vi "VIH HelpGen - Get Target HTML Filename.vi"(9 "Item File Path":path, 10 "Item Type":T1, 11 "HTML Filename in":string) -> (2 "same as source name":bool, 3 "HTML Fileame out":string)   [LabVIEW 2014]
doc: "::: VI Helpeks :::\nCopyright (c) 2000-2026 Konstantin Shifershteyn. All rights reserved."
uses:
  _VIH HelpGen - Palette.llb/VIH HelpGen Typedef - Palette - Item Type Enum.ctl
panel:
  # "VI Helpeks\nCopyright (c) 2012-2026 Konstantin Shifershteyn"
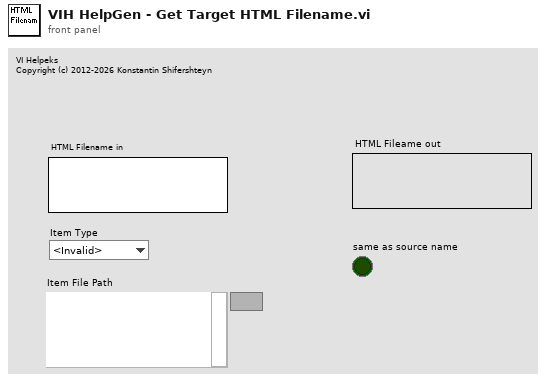
[diagram p1: front panel]
types:
  T1 = typedef "VIH HelpGen Typedef - Palette - Item Type Enum.ctl" = enum32{"<Invalid>", "<unknown>", "VI", "Menu", "LV Func", "Express VI", "Poly VI", "CTL", "HTML"}
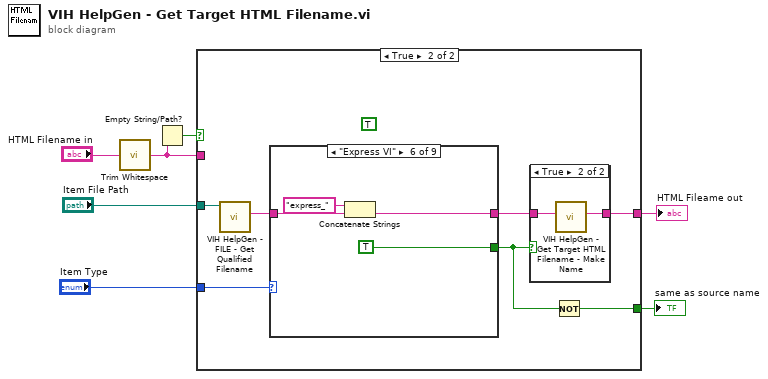
[diagram p0: block diagram]
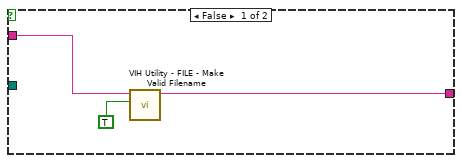
[diagram p2: hidden frame]
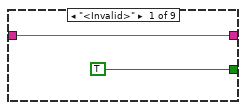
[diagram p4: hidden frame]
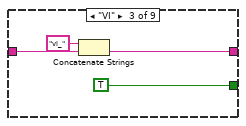
[diagram p6: hidden frame]
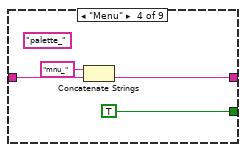
[diagram p7: hidden frame]
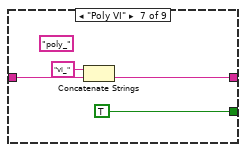
[diagram p9: hidden frame]
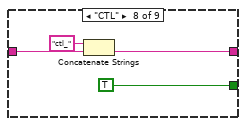
[diagram p10: hidden frame]
diagram:
  n1 = call <vilib>:"Trim Whitespace.vi"("string"="HTML Filename in") -> ("trimmed string"=w5:string)  [unwired: 1 in]
  n2 = Empty String/Path?(string/path=w5) -> (empty?=w6:bool)
  n3 = case shown="True" w6 {
    tunnel: [w9 w15] -> w2
    tunnel: w5 -> [w10 _]
    tunnel: "Item File Path" -> [_ w12]
    tunnel: "Item Type" -> [_ w17]
    tunnel: [_ w13] -> w1
    frame False {
      n4 = call "VIH Utility - FILE - Make Valid Filename.vi"("comply to CHM (F)"=TRUE, "File Name in"=w10) -> ("File Name out"=w9:string)  [unwired: 9 in]
    }
    frame True {
      (unwired) TRUE
      n5 = call "VIH HelpGen - FILE - Get Qualified Filename.vi"("File Path"=w12) -> ("Qualified name"=w11:string)  [unwired: 9 in, 1 out]
      n6 = case shown="\"Express VI\"" w17 {
        tunnel: w11 -> [w22 w23 w27 w31 w32 w36 w40 w44 w45]
        tunnel: [w22 w23 w26 w30 w32 w35 w39 w43 w45] -> w16
        tunnel: [TRUE _ TRUE TRUE _ TRUE TRUE TRUE _] -> w14
        frame "<Invalid>" {
        }
        frame "<unknown>" {
          # "don't change name of external file"
        }
        frame "VI" {
          n7 = Concatenate Strings("vi_" ("string"), w27) -> (w26:string)
        }
        frame "Menu" {
          (unwired) "palette_" ("string")
          n8 = Concatenate Strings("mnu_" ("string"), w31) -> (w30:string)
        }
        frame "LV Func" {
        }
        frame "Express VI" {
          n9 = Concatenate Strings("express_" ("string"), w36) -> (w35:string)
        }
        frame "Poly VI" {
          (unwired) "poly_" ("string")
          n10 = Concatenate Strings("vi_" ("string"), w40) -> (w39:string)
        }
        frame "CTL" {
          n11 = Concatenate Strings("ctl_" ("string"), w44) -> (w43:string)
        }
        frame "HTML" {
          # "don't change name of external file"
        }
      }
      n12 = case shown="True" w14 {
        tunnel: w16 -> [w18 w20]
        tunnel: [w18 w19] -> w15
        frame False {
        }
        frame True {
          n13 = call "VIH HelpGen - Get Target HTML Filename - Make Name.vi"("Item Filename"=w20) -> ("HTML Filename"=w19:string)  [unwired: 10 in]
        }
      }
      n14 = Not(x=w14) -> (.not. x?=w13:bool)
    }
  }
  "HTML Fileame out" <- w2
  "same as source name" <- w1
